vi "rotate_coin_planar.vi"(7 "pad Color":u32(colorbox)=7500402, 8 "error in (no error)":errorcluster, 10 "angle [rad]":sgl, 11 "image in":T1) -> (0 "error out":errorcluster, 3 "image out":T1)   [LabVIEW 2017, in "Image Processing Library.lvlib"]
uses:
  Image Processing Library.lvlib
  <vilib>/picture/picture.llb/imagedata.ctl
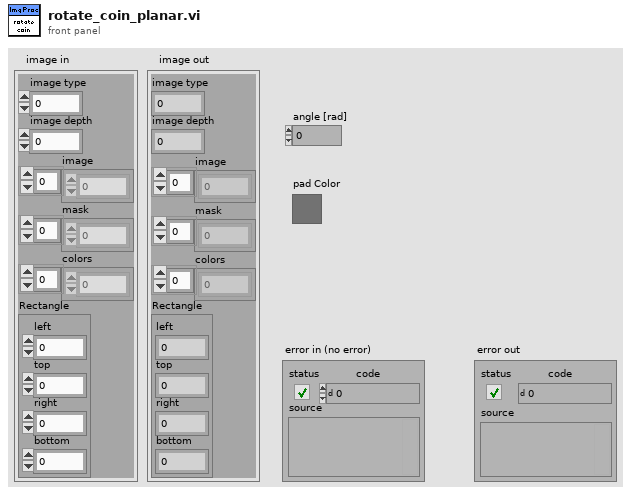
[diagram p1: front panel]
types:
  T1 = typedef "imagedata.ctl" = cluster{"image type":i32, "image depth":i32, "image":u8[], "mask":u8[], "colors":u32[], "Rectangle":cluster{"left":i16, "top":i16, "right":i16, "bottom":i16}}
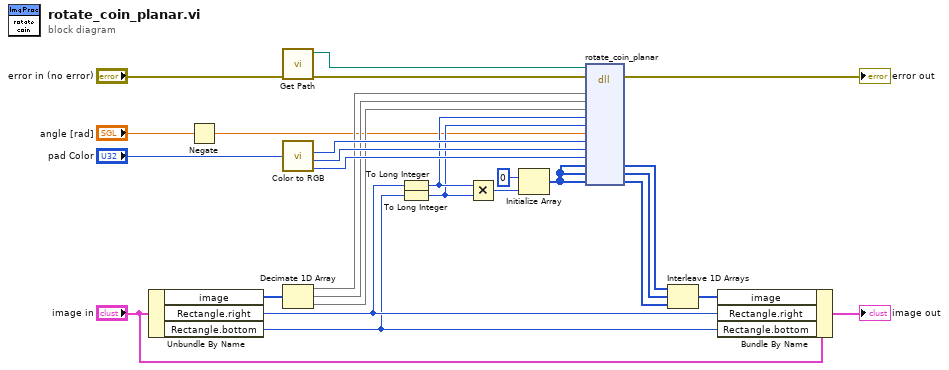
[diagram p0: block diagram]
diagram:
  n1 = Unbundle By Name("image in") -> ("image"=w16:u8[], "Rectangle.right"=w5:i16, "Rectangle.bottom"=w4:i16)
  n2 = Negate(x="angle [rad]") -> (-x=w1:sgl)
  n3 = call "Get Path.vi"("error in (no error)"="error in (no error)") -> ("error out"=w26:errorcluster, "Library Path"=w25:path)  [unwired: 9 in]
  n4 = call <vilib>:"Color to RGB.vi"("Color"="pad Color") -> ("R"=w22:u8, "G"=w21:u8, "B"=w20:u8)  [unwired: 1 out]
  n5 = Decimate 1D Array(w16) -> (w15:u8[], w14:u8[], w13:u8[])
  n6 = To Long Integer(number=w5) -> (32bit integer=w3:i32)
  n7 = To Long Integer(number=w4) -> (32bit integer=w2:i32)
  n8 = Multiply(x=w3, y=w2) -> (x*y=w19:i32)
  n9 = Initialize Array(u8 0 ("element"), w19) -> (w17:u8[])
  n10 = dll-call lib="C:/Users/IvanLis-Win10/Desktop/LabVIEW/Coin Detector/Project_2018/image_processing/windows_x64/image_processing.dll" fn="rotate_coin_planar"(path in=w25, error in=w26, "in_r"=w15, "in_g"=w14, "in_b"=w13, "orig_w"=w3, "orig_h"=w2, "angle"=w1, "pad_r"=w22, "pad_g"=w21, "pad_b"=w20, "out_r"=w17, "out_g"=w17, "out_b"=w17) -> (error out=→"error out":errorcluster, "out_r"=w12:u8[], "out_g"=w11:u8[], "out_b"=w10:u8[])  [unwired: 11 in, 1 out]
  n11 = Interleave 1D Arrays(w12, w11, w10) -> (w9:u8[])
  n12 = Bundle By Name(cluster="image in", "image"=w9, "Rectangle.right"=w5, "Rectangle.bottom"=w4) -> (→"image out":T1)
